vi "CreateClass.vi"(0 "ClassWriterGOOP400.lvclass":refnum<class "ClassWriterGOOP400.lvclass">, 1 "ProjectTreePosition(String or Project Item Ref)":variant, 2 "CreateClassData":T1, 5 "error in (no error)":errorcluster, 6 "KeepLvClassRefOpen(False)":bool, 7 "HeaderToApply (take from VIRef or /use 2D-8bit header, Ignored if not wired)":variant) -> (14 "ClassWriterGOOP400.lvclass":refnum<class "ClassWriterGOOP400.lvclass">, 15 "LVClassLibraryRefnum":refnum<vi>, 16 "TemplateVersionUsed":string, 19 "error out":errorcluster)   [LabVIEW 2020, in "ClassWriterGOOP400.lvclass"]
uses:
  ClassWriterGOOP400.lvclass
  Provider_BaseClassInterface/CreateClassData.ctl
  Common/LvClass_class/GDSLvCLass_ClassSettingsType.ctl
  Common/LvClass_class/GDSLvClass_PlugIn.ctl
  Common/LvClass_class/GDSLvClass_PlugInTypes.ctl
  EndevoG4ProviderName.ctl
  Provider_BaseClassInterface/ClassWriter_class/ClassWriter.lvclass
  Provider_LvNativeClass/ClassWriterNative_class/ClassWriterNative.lvclass
  Common/InterfaceLibrary/InterfaceLibrary.lvlib
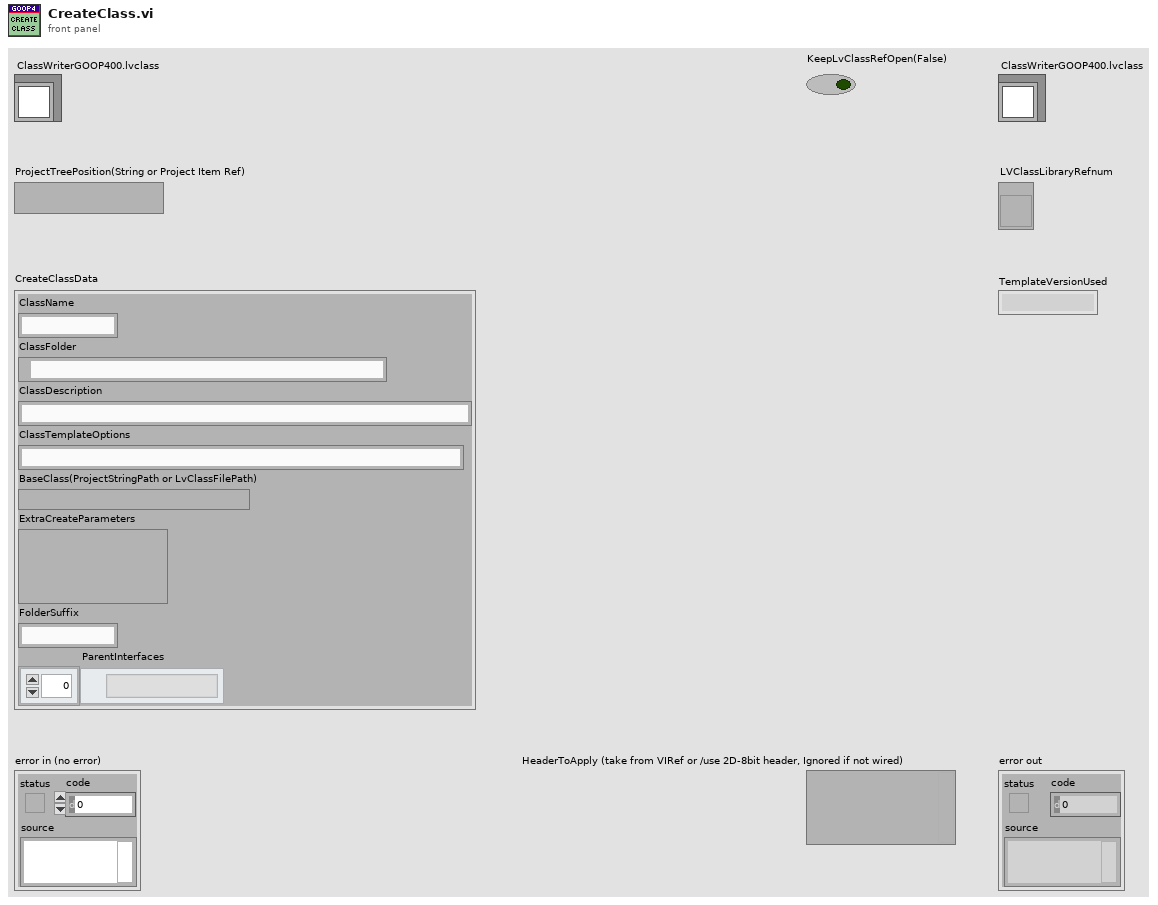
[diagram p1: front panel]
types:
  T1 = typedef "ClassWriter.lvclass/CreateClassData.ctl" = cluster{"ClassName":string, "ClassFolder":path, "ClassDescription":string, "ClassTemplateOptions":string, "BaseClass(ProjectStringPath or LvClassFilePath)":variant, "ExtraCreateParameters":variant, "FolderSuffix":string, "ParentInterfaces":path[]}
  T2 = typedef "GDSLvCLass_ClassSettingsType.ctl" = cluster{"ClassProviderName":string, "ClassTemplateUsed":string, "ClassTemplateVersion":string, "ClassDescription":string, "PlugIns":T3[], "ConnectorPanePattern":string}
  T3 = typedef "GDSLvClass_PlugIn.ctl" = cluster{"Type":T4, "ID":string, "Version":string, "Path":path, "Name":string, "Data":variant}
  T4 = typedef "GDSLvClass_PlugInTypes.ctl" = enum16{"DesignPattern", "MethodTypes"}
  T5 = cluster{"SubClass":bool, "ClassTemplateFiles":path[], "ClassName":string, "ClassFolder":path, "VIs":refnum<vi>[], "TemplateFolder":path, "ViSubDirs":string[], "TemplateName":string, "BaseClassFolder":path, "RootBaseClassFolder":path, "LvClassPath":path, "ClassRefnum":refnum<vi>, "ProjectRefnum":refnum<vi>, "LvClassFolderPath":path, "BaseClassName":string, "ClassItems":refnum<vi>[], "ViLocked":bool[], "ProjectItemOwner":refnum<vi>, "DeleteFiles":path[], "VIsBefore":refnum<vi>[], "BaseClassPath":path, "BaseConstructorBase":path, "TemplBaseConstructorBase":path, "TemplatePath":path, "TemplateVersion":string, "TemplateParentClass":refnum<vi>, "App":refnum<vi>, "Parent Class":refnum<vi>, "ParentVIs":refnum<vi>[], "TempClass":refnum<vi>, "ClassSettings":T2}
  T6 = typedef "EndevoG4ProviderName.ctl" = enum16{"EndevoGOOP400"}
  T7 = enum32{"invalid scope", "public", "private", "protected"}
  T8 = enum32{"invalid lock state", "Not Locked", "Locked (No Password)", "Password-protected"}
  T9 = typedef "ClassWriter.lvclass/TemplateSettings.ctl" = cluster{"CommonClassTemplate":bool, "DynamicDispatch":enum8{"False", "True", "Mixed"}, "MustOverride":enum8{"False", "True", "Mixed"}, "MustCallParent":enum8{"False", "True", "Mixed"}, "OnlyNormalMethod":bool, "OnlyPublic":bool}
  T10 = typedef "Scripting_ConnectorPanePatternType.ctl" = u16
  T11 = typedef "GOOP400_Options.ctl" = cluster{"FlatFolderStructure":bool}
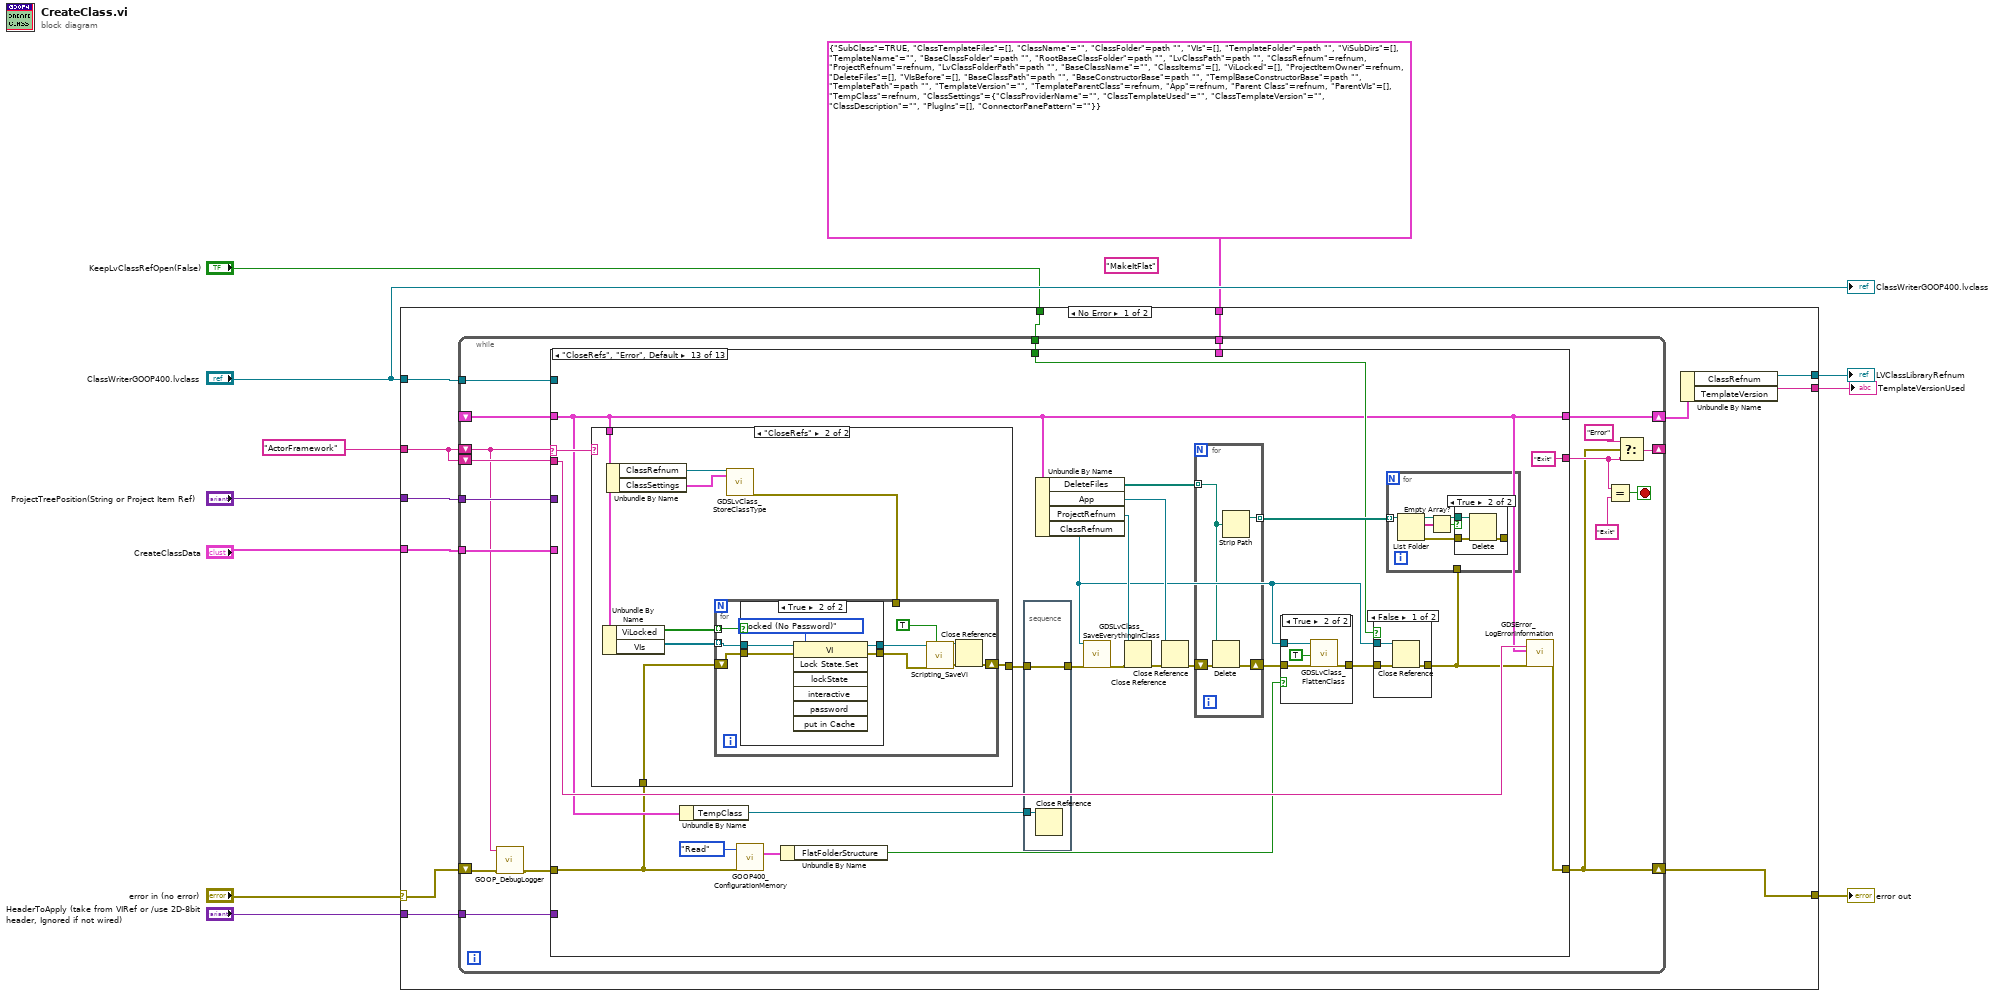
[diagram p0: block diagram]
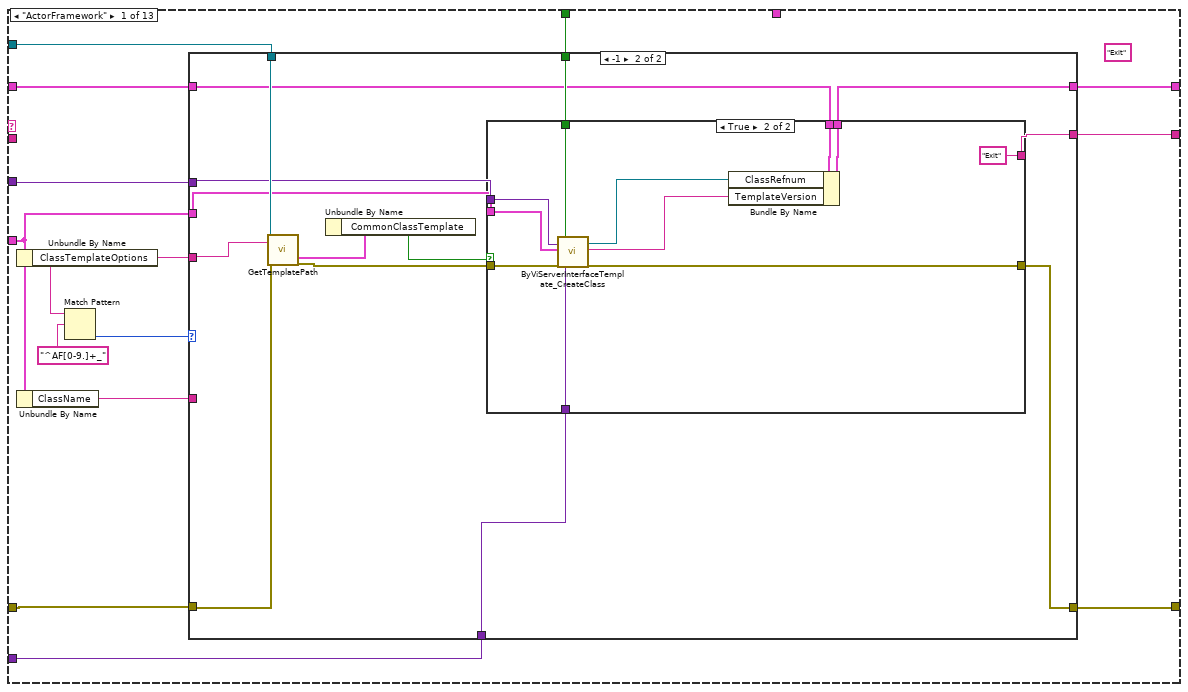
[diagram p2: hidden frame]
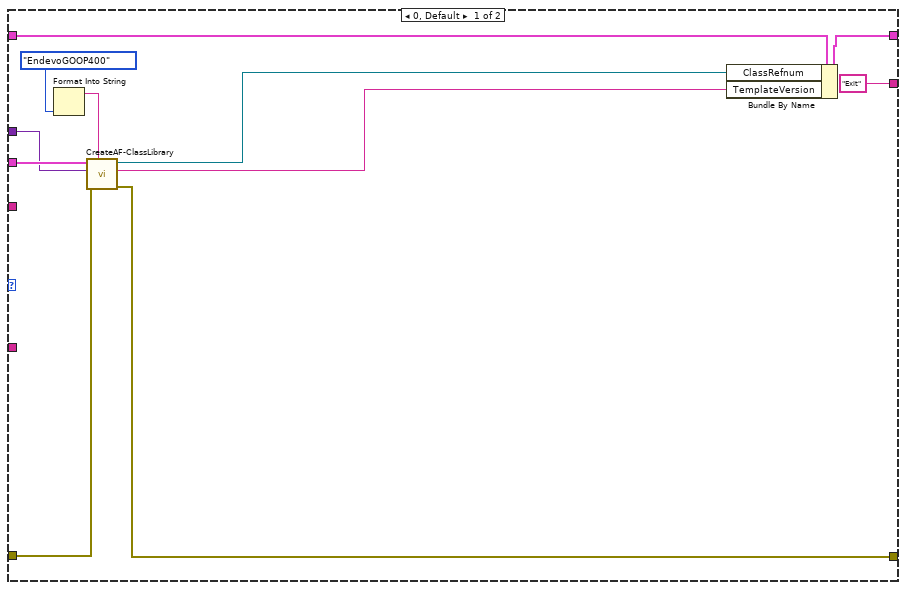
[diagram p3: hidden frame]
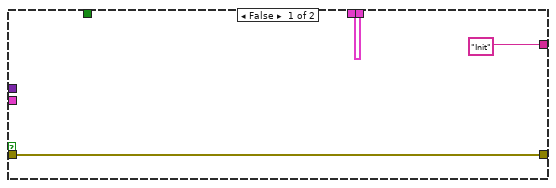
[diagram p4: hidden frame]
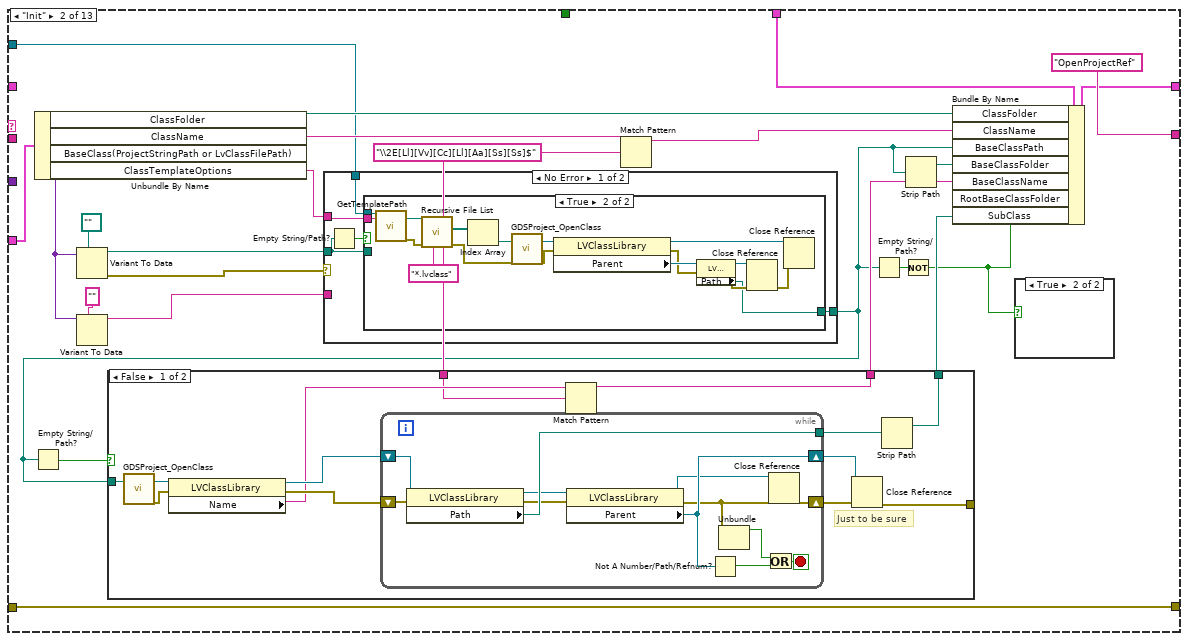
[diagram p5: hidden frame]
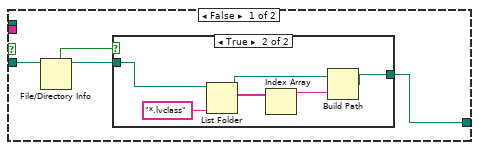
[diagram p6: hidden frame]
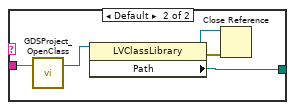
[diagram p9: hidden frame]
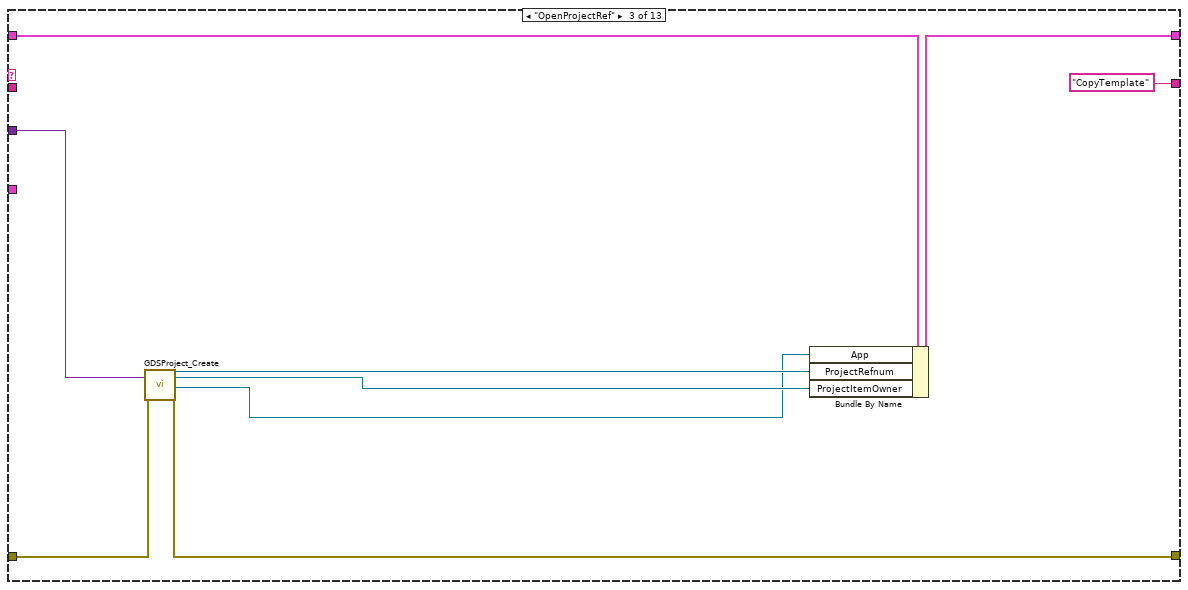
[diagram p12: hidden frame]
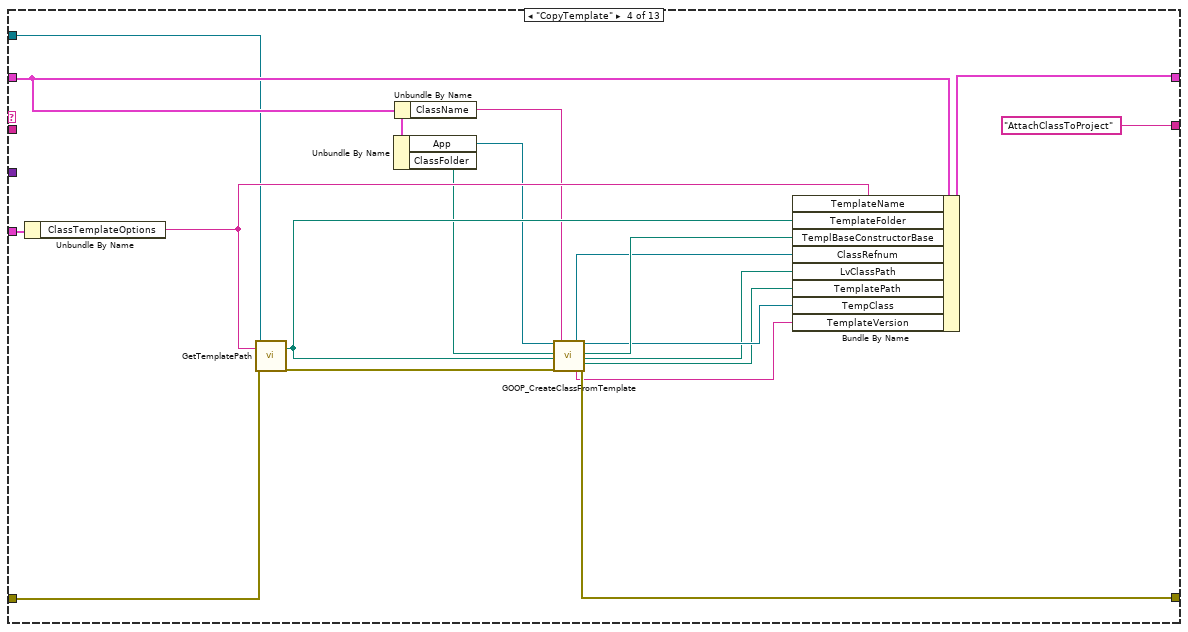
[diagram p13: hidden frame]
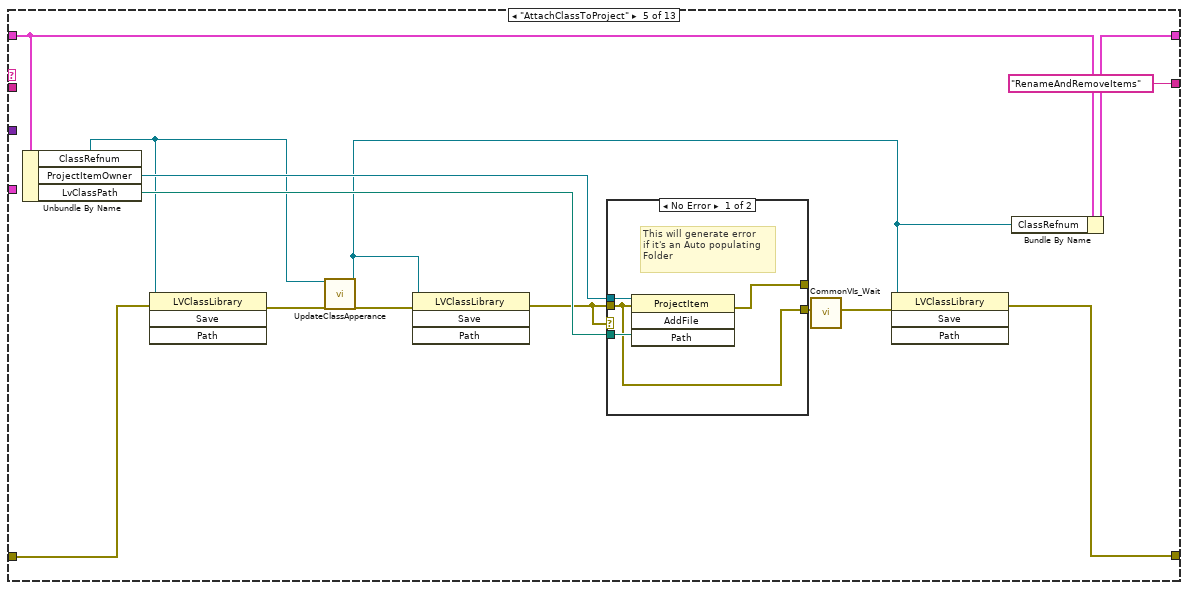
[diagram p14: hidden frame]
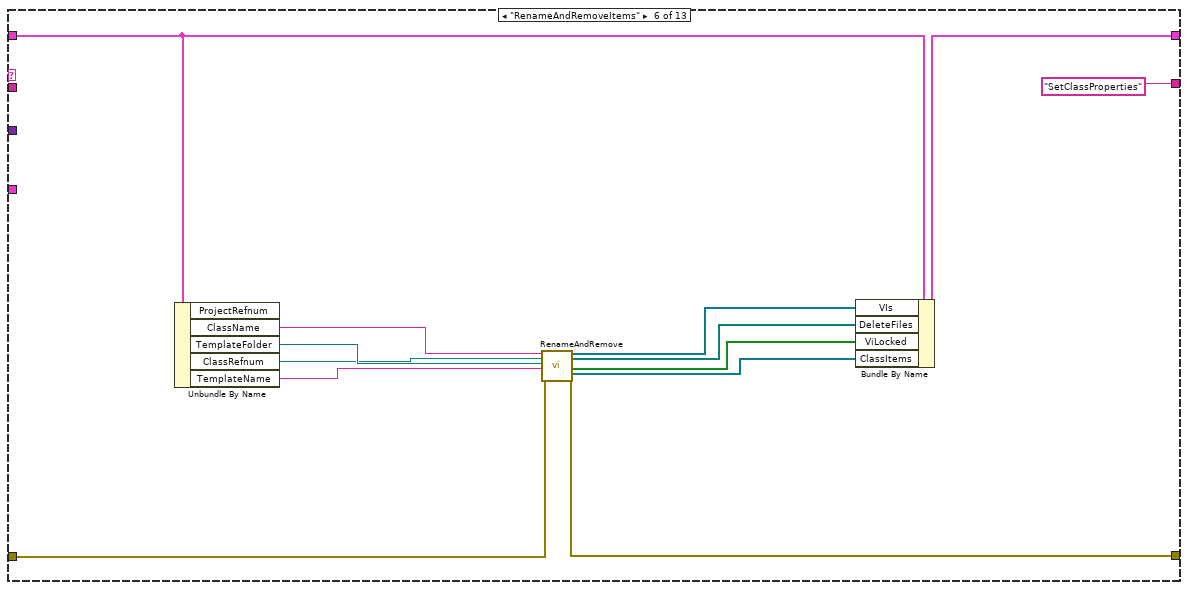
[diagram p16: hidden frame]
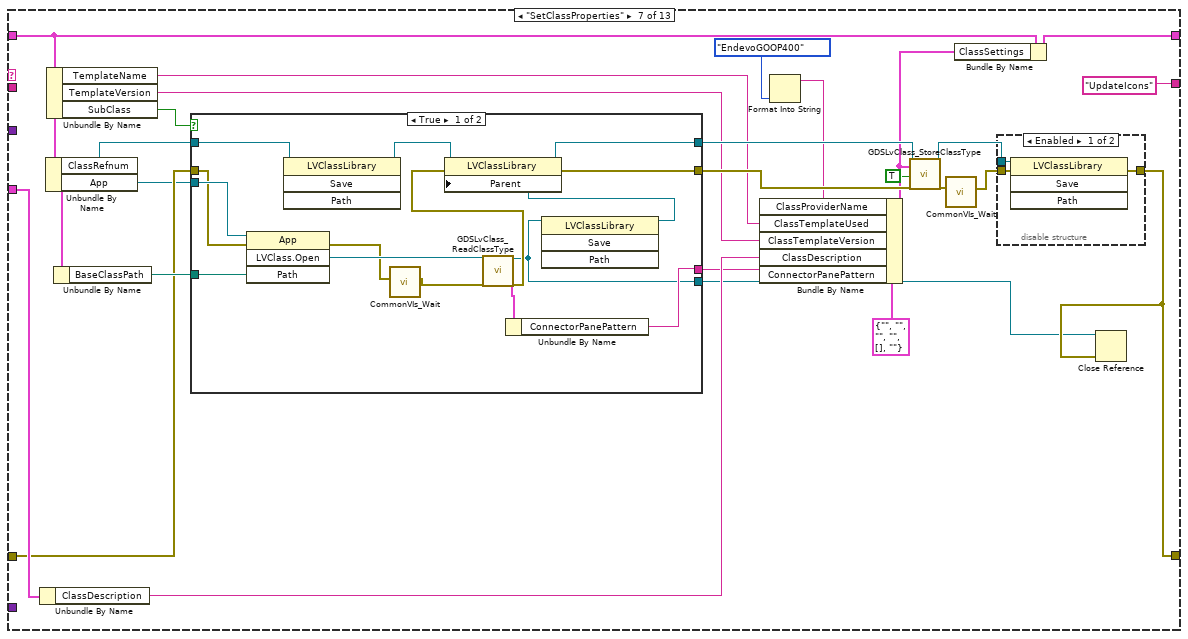
[diagram p17: hidden frame]
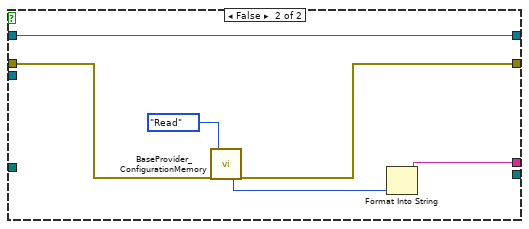
[diagram p19: hidden frame]
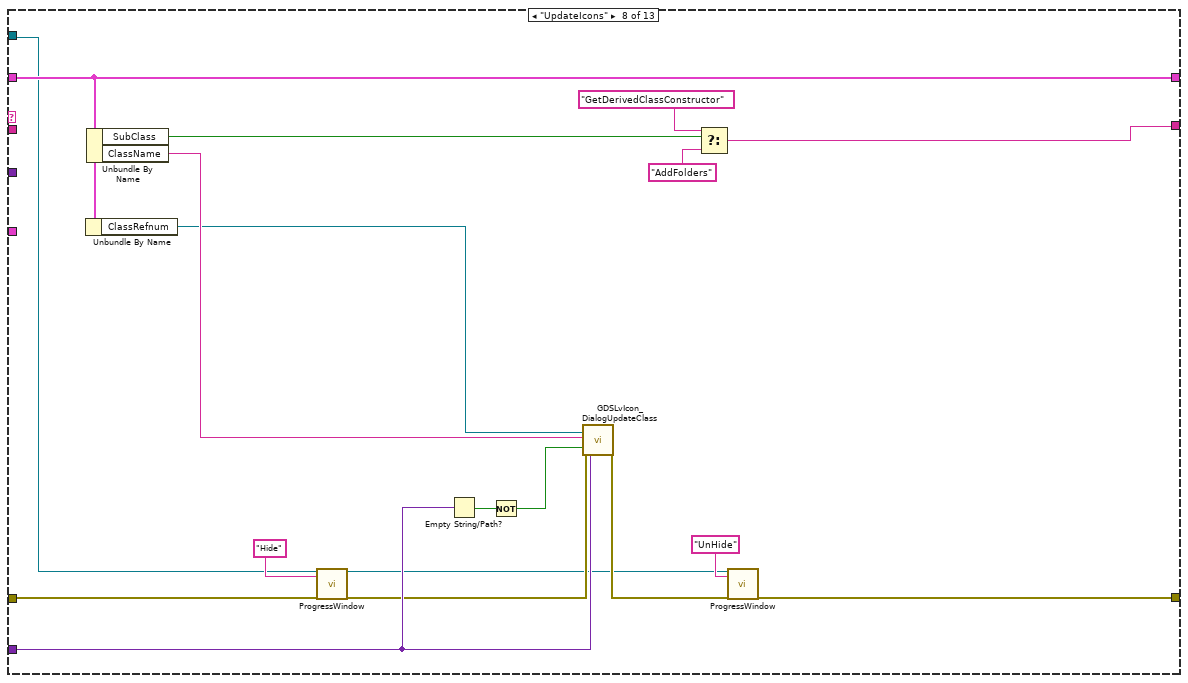
[diagram p20: hidden frame]
diagram:
  (unwired) "MakeItFlat"
  n1 = case shown="No Error" "error in (no error)" {
    selector: "error in (no error)" -> [w13 w610]
    tunnel: [w23 w610] -> w11
    tunnel: "ProjectTreePosition(String or Project Item Ref)" -> [w22 _]
    tunnel: "CreateClassData" -> [w21 _]
    tunnel: "ClassWriterGOOP400.lvclass" -> [w20 _]
    tunnel: "HeaderToApply (take from VIRef or /use 2D-8bit header, Ignored if not wired)" -> [w19 _]
    tunnel: "KeepLvClassRefOpen(False)" -> [w18 _]
    tunnel: [w17 _] -> w4
    tunnel: [w16 _] -> w3
    tunnel: T5 {"SubClass"=TRUE, "ClassTemplateFiles"=[], "ClassName"="", "ClassFolder"=path "", "VIs"=[], "TemplateFolder"=path "", "ViSubDirs"=[], "TemplateName"="", "BaseClassFolder"=path "", "RootBaseClassFolder"=path "", "LvClassPath"=path "", "ClassRefnum"=refnum, "ProjectRefnum"=refnum, "LvClassFolderPath"=path "", "BaseClassName"="", "ClassItems"=[], "ViLocked"=[], "ProjectItemOwner"=refnum, "DeleteFiles"=[], "VIsBefore"=[], "BaseClassPath"=path "", "BaseConstructorBase"=path "", "TemplBaseConstructorBase"=path "", "TemplatePath"=path "", "TemplateVersion"="", "TemplateParentClass"=refnum, "App"=refnum, "Parent Class"=refnum, "ParentVIs"=[], "TempClass"=refnum, "ClassSettings"={"ClassProviderName"="", "ClassTemplateUsed"="", "ClassTemplateVersion"="", "ClassDescription"="", "PlugIns"=[], "ConnectorPanePattern"=""}} ("output cluster") -> [w15 _]
    tunnel: "ActorFramework" -> [w12 _]
    frame No Error {
      n2 = while {
        shift-right: [w33] -> w23
        shift-left: w13 -> [w26]
        shift-right: [w37] -> _
        shift-left: w12 -> [w24]
        shift-right: [w40] -> w14
        shift-left: _ -> [w41]
        tunnel: w15 -> [w35]
        tunnel: w22 -> [w32]
        tunnel: w21 -> [w31]
        tunnel: w20 -> [w30]
        shift-left: w12 -> [w29]
        tunnel: w19 -> [w28]
        tunnel: w18 -> [w27]
        stop <- w38 stop-if-true
        n3 = call "GOOP_DebugLogger.vi"("error in (no error)"=w26, "State"=w24) -> ("error out"=w25:errorcluster)  [unwired: 7 in, 2 out]
        n4 = case shown="\"CloseRefs\", \"Error\", Default" w24 {
          selector: w24 -> [_ _ _ _ _ _ _ _ _ _ _ _ w558]
          tunnel: w41 -> [w55 _ w190 w208 w223 w238 w256 w306 w328 w337 w450 w516 w547]
          tunnel: [w54 w115 w189 w210 w222 w240 w245 w306 w329 w337 w450 w516 w547] -> w40
          tunnel: w25 -> [w50 w118 w188 w204 w217 w235 w257 w299 w325 w351 w471 w518 w542]
          tunnel: [w49 w118 w186 w199 w213 w236 w247 w296 w311 w335 w451 w519 w556] -> w33
          tunnel: [w53 "OpenProjectRef" "CopyTemplate" "AttachClassToProject" "RenameAndRemoveItems" "SetClassProperties" "UpdateIcons" w308 "UpdateVIs" ("t") "AddFolders" "AddFolders" "CloseRefs" "Exit"] -> w34
          tunnel: w35 -> [_ w112 _ _ _ _ _ _ _ _ _ _ _]
          tunnel: w32 -> [w48 _ w187 _ _ _ _ _ _ _ _ _ _]
          tunnel: w31 -> [w46 w111 _ w207 _ _ w263 _ _ _ _ w507 _]
          tunnel: w30 -> [w44 w97 _ w205 _ _ _ w293 _ _ _ _ _]
          tunnel: w29 -> [_ _ _ _ _ _ _ _ _ _ _ _ w555]
          tunnel: w28 -> [w42 _ _ _ _ _ _ w304 _ _ _ _ _]
          tunnel: w27 -> [w43 _ _ _ _ _ _ _ _ _ _ _ w552]
          frame "ActorFramework" {
            (unwired) "Exit"
            n5 = Unbundle By Name(w46) -> ("ClassTemplateOptions"=w47:string)
            n6 = Unbundle By Name(w46) -> ("ClassName"=w45:string)
            n7 = Match Pattern(string=w47, regular expression="^AF[0-9.]+_") -> (offset past match=w51:i32)  [unwired: 1 in, 3 out]
            n8 = case shown="-1" w51 {
              tunnel: w55 -> [w66 w73]
              tunnel: [w65 w72] -> w54
              tunnel: ["Exit" w80] -> w53
              tunnel: w46 -> [w63 w70]
              tunnel: w50 -> [w62 w79]
              tunnel: [w61 w75] -> w49
              tunnel: w48 -> [w58 w71]
              tunnel: w47 -> [_ w77]
              tunnel: w45 -> [_ _]
              tunnel: w44 -> [_ w78]
              tunnel: w43 -> [_ w74]
              tunnel: w42 -> [_ w69]
              frame 0, Default {
                n9 = Format Into String(EndevoG4ProviderName."EndevoGOOP400" ("ProviderName")) -> (resulting string=w60:string)  [unwired: 3 in, 1 out]
                n10 = call "CreateAF-ClassLibrary.vi"("Providername"=w60, "error in (no error)"=w62, "ProjectTreePosition(String or Project Item Ref)"=w58, "CreateClassData"=w63) -> ("error out"=w61:errorcluster, "TemplateVersionUsed"=w59:string, "LVClassLibraryRefnum"=w56:refnum<vi>)  [unwired: 5 in]
                n11 = Bundle By Name(cluster=w66, "ClassRefnum"=w56, "TemplateVersion"=w59) -> (w65:T5)
              }
              frame -1 {
                n12 = call-dynamic "GetTemplatePath.vi"("reference in"=w78, "ClassTemplateSubDirectory"=w77, "error in (no error)"=w79) -> ("TemplateSettings"=w68:T9, "error out"=w76:errorcluster)  [unwired: 12 in, 3 out]
                n13 = Unbundle By Name(w68) -> ("CommonClassTemplate"=w67:bool)
                n14 = case shown="True" w67 {
                  tunnel: ["Init" "Exit"] -> w80
                  tunnel: w76 -> [w82 w91]
                  tunnel: [w82 w90] -> w75
                  tunnel: w74 -> [_ w89]
                  tunnel: w73 -> [w81 w88]
                  tunnel: [w81 w87] -> w72
                  tunnel: w71 -> [_ w86]
                  tunnel: w70 -> [_ w85]
                  tunnel: w69 -> [_ w84]
                  frame False {
                  }
                  frame True {
                    n15 = call "ByViServerInterfaceTemplate_CreateClass.vi"("ProjectTreePosition(String or Project Item Ref)"=w86, "CreateClassData"=w85, "error in (no error)"=w91, "KeepLvClassRefOpen(False)"=w89, "HeaderToApply (take from VIRef or /use 2D-8bit header, Ignored if not wired)"=w84) -> ("LVClassLibraryRefnum"=w93:refnum<vi>, "TemplateVersionUsed"=w92:string, "error out"=w90:errorcluster)  [unwired: 12 in]
                    n16 = Bundle By Name(cluster=w88, "ClassRefnum"=w93, "TemplateVersion"=w92) -> (w87:T5)
                  }
                }
              }
            }
          }
          frame "Init" {
            w108 = "\\2E[Ll][Vv][Cc][Ll][Aa][Ss][Ss]$" ("regular expression")
            n17 = Unbundle By Name(w111) -> ("ClassFolder"=w105:path, "ClassName"=w104:string, "BaseClass(ProjectStringPath or LvClassFilePath)"=w110:variant, "ClassTemplateOptions"=w96:string)
            n18 = Variant To Data(type=path "" ("path"), Variant=w110) -> (data=w100:path, error out=w99:errorcluster)  [unwired: 1 in]
            n19 = Variant To Data(type="" ("regular expression"), Variant=w110) -> (data=w98:string)  [unwired: 1 in, 1 out]
            n20 = case shown="No Error" w99 {
              tunnel: [w123 w152] -> w95
              tunnel: w98 -> [_ w153]
              tunnel: w100 -> [w122 _]
              tunnel: w96 -> [w119 _]
              tunnel: w97 -> [w120 _]
              frame No Error {
                n21 = Empty String/Path?(string/path=w122) -> (empty?=w121:bool)
                n22 = case shown="True" w121 {
                  tunnel: [w127 w135] -> w123
                  tunnel: w122 -> [w124 _]
                  tunnel: w120 -> [_ w137]
                  tunnel: w119 -> [_ w136]
                  frame False {
                    n23 = File/Directory Info(path=w124) -> (path out=w125:path, directory=w126:bool)  [unwired: 1 in, 5 out]
                    n24 = case shown="True" w126 {
                      tunnel: [w128 w130] -> w127
                      tunnel: w125 -> [w128 w129]
                      frame False {
                      }
                      frame True {
                        n25 = List Folder(path=w129, pattern="*.lvclass") -> (path out=w131:path, filenames=w133:string[])  [unwired: 2 in, 2 out]
                        n26 = Index Array(array=w133) -> (element=w132:string)  [unwired: 1 in]
                        n27 = Build Path(base path=w131, name or relative path=w132) -> (appended path=w130:path)
                      }
                    }
                  }
                  frame True {
                    n28 = call-dynamic "GetTemplatePath.vi"("reference in"=w137, "ClassTemplateSubDirectory"=w136) -> ("FolderPathOut"=w149:path, "error out"=w139:errorcluster)  [unwired: 13 in, 3 out]
                    n29 = call <vilib>:"Recursive File List.vi"("pattern"="*.lvclass", "error in (no error)"=w139, "Folder Path"=w149) -> ("error out"=w138:errorcluster, "All Files in Dir"=w150:path[])  [unwired: 4 in, 3 out]
                    n30 = Index Array(array=w150) -> (element=w148:path)  [unwired: 1 in]
                    n31 = call "GDSProject_OpenClass.vi"("ClassPath(FilePath/ProjectTreePath/LvCLassRef)"=w148, "error IO"=w138) -> ("LVClass.Open"=w146:refnum<vi>, "error out"=w147:errorcluster)  [unwired: 15 in, 1 out]
                    n32 = property class="LVClassLibrary"(reference=w146, error in=w147) -> (reference out=w140:refnum<vi>, error out=w144:errorcluster, "Parent"=w145:refnum<vi>)
                    n33 = property class="LVClassLibrary"(reference=w145, error in=w144) -> (reference out=w142:refnum<vi>, error out=w143:errorcluster, "Path"=w135:path)
                    n34 = Close Reference(reference=w142, error in (no error)=w143) -> (error out=w141:errorcluster)
                    n35 = Close Reference(reference=w140, error in (no error)=w141) -> ()  [unwired: 1 out]
                  }
                }
              }
              frame Error {
                n36 = case shown="\"\"" w153 {
                  tunnel: w153 -> [_ w158]
                  tunnel: [_ w154] -> w152
                  frame "" {
                  }
                  frame Default {
                    n37 = call "GDSProject_OpenClass.vi"("ClassPath(FilePath/ProjectTreePath/LvCLassRef)"=w158) -> ("LVClass.Open"=w157:refnum<vi>)  [unwired: 16 in, 2 out]
                    n38 = property class="LVClassLibrary"(reference=w157) -> (reference out=w155:refnum<vi>, error out=w156:errorcluster, "Path"=w154:path)  [unwired: 1 in]
                    n39 = Close Reference(reference=w155, error in (no error)=w156) -> ()  [unwired: 1 out]
                  }
                }
              }
            }
            n40 = Empty String/Path?(string/path=w95) -> (empty?=w106:bool)
            n41 = case shown="False" w106 {
              tunnel: [w168 _] -> w109
              tunnel: w108 -> [w162 _]
              tunnel: [w161 _] -> w107
              tunnel: w95 -> [w160 _]
              tunnel: [w159 _] -> _
              frame False {
                # "Just to be sure"
                n42 = call "GDSProject_OpenClass.vi"("ClassPath(FilePath/ProjectTreePath/LvCLassRef)"=w160) -> ("LVClass.Open"=w165:refnum<vi>, "error out"=w167:errorcluster)  [unwired: 16 in, 1 out]
                n43 = property class="LVClassLibrary"(reference=w165, error in=w167) -> (reference out=w164:refnum<vi>, error out=w166:errorcluster, "Name"=w163:string)
                n44 = while {
                  shift-right: [w179] -> w171
                  shift-left: w166 -> [w174]
                  shift-right: [w180] -> w170
                  shift-left: w164 -> [w182]
                  tunnel: [w181] -> w169
                  stop <- w176 stop-if-true
                  n45 = property class="LVClassLibrary"(reference=w182, error in=w174) -> (reference out=w172:refnum<vi>, error out=w173:errorcluster, "Path"=w181:path)
                  n46 = property class="LVClassLibrary"(reference=w172, error in=w173) -> (reference out=w175:refnum<vi>, error out=w179:errorcluster, "Parent"=w180:refnum<vi>)
                  n47 = Not A Number/Path/Refnum?(number/path/refnum=w180) -> (NaN/Path/Refnum?=w177:bool)
                  n48 = Unbundle(w179) -> ("status"=w178:bool)  [unwired: 2 out]
                  n49 = Or(x=w178, y=w177) -> (x .or. y?=w176:bool)
                  n50 = Close Reference(reference=w175) -> ()  [unwired: 1 in, 1 out]
                }
                n51 = Match Pattern(string=w163, regular expression=w162) -> (before substring=w161:string)  [unwired: 1 in, 3 out]
                n52 = Close Reference(reference=w170, error in (no error)=w171) -> (error out=w159:errorcluster)
                n53 = Strip Path(path=w169) -> (stripped path=w168:path)  [unwired: 1 out]
              }
              frame True {
              }
            }
            n54 = Match Pattern(string=w104, regular expression=w108) -> (before substring=w116:string)  [unwired: 1 in, 3 out]
            n55 = Empty String/Path?(string/path=w95) -> (empty?=w102:bool)
            n56 = Not(x=w102) -> (.not. x?=w101:bool)
            n57 = Strip Path(path=w95) -> (stripped path=w103:path)  [unwired: 1 out]
            n58 = Bundle By Name(cluster=w112, "ClassFolder"=w105, "ClassName"=w116, "BaseClassPath"=w95, "BaseClassFolder"=w103, "BaseClassName"=w107, "RootBaseClassFolder"=w109, "SubClass"=w101) -> (w115:T5)
            n59 = case shown="True" w101 {
              frame False {
              }
              frame True {
              }
            }
          }
          frame "OpenProjectRef" {
            n60 = call "GDSProject_Create.vi"("ProjectTreePosition(String or Project Item Ref)"=w187, "error in (no error)"=w188) -> ("Project Refnum"=w184:refnum<vi>, "Project Item"=w185:refnum<vi>, "App"=w183:refnum<vi>, "error out"=w186:errorcluster)  [unwired: 13 in, 1 out]
            n61 = Bundle By Name(cluster=w190, "App"=w183, "ProjectRefnum"=w184, "ProjectItemOwner"=w185) -> (w189:T5)
          }
          frame "CopyTemplate" {
            n62 = Unbundle By Name(w207) -> ("ClassTemplateOptions"=w206:string)
            n63 = call-dynamic "GetTemplatePath.vi"("reference in"=w205, "ClassTemplateSubDirectory"=w206, "error in (no error)"=w204) -> ("FolderPathOut"=w202:path, "error out"=w203:errorcluster)  [unwired: 12 in, 3 out]
            n64 = Unbundle By Name(w208) -> ("App"=w200:refnum<vi>, "ClassFolder"=w196:path)
            n65 = Unbundle By Name(w208) -> ("ClassName"=w192:string)
            n66 = call "GOOP_CreateClassFromTemplate.vi"("Application in"=w200, "ClassFolder"=w196, "TeplateClassFolder"=w202, "error in (no error)"=w203, "ClassName"=w192) -> ("NewClassRef"=w193:refnum<vi>, "TemplateClassVersionString"=w194:string, "TemplateClassRef"=w198:refnum<vi>, "TemplateClassConstructorPath(*Create, *Init)"=w201:path, "NewClassPath"=w197:path, "TemplateClassPath"=w195:path, "error out"=w199:errorcluster)  [unwired: 7 in, 1 out]
            n67 = Bundle By Name(cluster=w208, "TemplateName"=w206, "TemplateFolder"=w202, "TemplBaseConstructorBase"=w201, "ClassRefnum"=w193, "LvClassPath"=w197, "TemplatePath"=w195, "TempClass"=w198, "TemplateVersion"=w194) -> (w210:T5)
          }
          frame "AttachClassToProject" {
            n68 = Unbundle By Name(w223) -> ("ClassRefnum"=w216:refnum<vi>, "ProjectItemOwner"=w224:refnum<vi>, "LvClassPath"=w220:path)
            n69 = invoke class="LVClassLibrary" method="Save"(reference=w216, error in=w217) -> (error out=w218:errorcluster)  [unwired: 2 in, 3 out]
            n70 = call "UpdateClassApperance.vi"("ClassRefIn"=w216, "error in (no error)"=w218) -> ("ClassRefOut"=w211:refnum<vi>, "error out"=w215:errorcluster)  [unwired: 16 in]
            n71 = invoke class="LVClassLibrary" method="Save"(reference=w211, error in=w215) -> (error out=w212:errorcluster)  [unwired: 2 in, 3 out]
            n72 = case shown="No Error" w212 {
              tunnel: w224 -> [w228 _]
              tunnel: w220 -> [w227 _]
              tunnel: [w226 w229] -> w219
              tunnel: w212 -> [w226 w229]
              tunnel: [w225 _] -> _
              frame No Error {
                # "This will generate error\nif it's an Auto populating\nFolder"
                n73 = invoke class="ProjectItem" method="AddFile"(reference=w228, error in=w226, "Path"=w227) -> (error out=w225:errorcluster)  [unwired: 1 in, 3 out]
              }
              frame Error {
              }
            }
            n74 = call "CommonVIs_Wait.vi"("error in"=w219) -> ("error out"=w214:errorcluster)  [unwired: 9 in]
            n75 = invoke class="LVClassLibrary" method="Save"(reference=w211, error in=w214) -> (error out=w213:errorcluster)  [unwired: 2 in, 3 out]
            n76 = Bundle By Name(cluster=w223, "ClassRefnum"=w211) -> (w222:T5)
          }
          frame "RenameAndRemoveItems" {
            n77 = Unbundle By Name(w238) -> ("ClassName"=w242:string, "TemplateFolder"=w239:path, "ClassRefnum"=w237:refnum<vi>, "TemplateName"=w230:string)  [unwired: 1 out]
            n78 = call "RenameAndRemove.vi"("ClassName"=w242, "ClassRefnum"=w237, "TemplateFolder"=w239, "TemplateName"=w230, "error in"=w235) -> ("ViRefsOut"=w241:refnum<vi>[], "DeleteFiles"=w234:path[], "ItemLocked"=w233:bool[], "Items"=w232:refnum<vi>[], "error out"=w236:errorcluster)  [unwired: 10 in]
            n79 = Bundle By Name(cluster=w238, "VIs"=w241, "DeleteFiles"=w234, "ViLocked"=w233, "ClassItems"=w232) -> (w240:T5)
          }
          frame "SetClassProperties" {
            n80 = Unbundle By Name(w263) -> ("ClassDescription"=w260:string)
            n81 = Unbundle By Name(w256) -> ("ClassRefnum"=w258:refnum<vi>, "App"=w252:refnum<vi>)
            n82 = Unbundle By Name(w256) -> ("TemplateName"=w259:string, "TemplateVersion"=w253:string, "SubClass"=w267:bool)
            n83 = Unbundle By Name(w256) -> ("BaseClassPath"=w266:path)
            n84 = case shown="True" w267 {
              tunnel: w258 -> [w275 w292]
              tunnel: [w286 w292] -> w265
              tunnel: w257 -> [w279 w289]
              tunnel: [w285 w288] -> w264
              tunnel: w266 -> [w284 _]
              tunnel: w252 -> [w280 _]
              tunnel: [w281 w290] -> w251
              tunnel: [w273 _] -> w246
              frame True {
                n85 = invoke class="App" method="LVClass.Open"(reference=w280, error in=w279, "Path"=w284) -> (error out=w278:errorcluster, "LVClass.Open"=w283:refnum<vi>)  [unwired: 1 in, 2 out]
                n86 = invoke class="LVClassLibrary" method="Save"(reference=w275) -> (reference out=w274:refnum<vi>)  [unwired: 3 in, 3 out]
                n87 = call "CommonVIs_Wait.vi"("error in"=w278) -> ("error out"=w277:errorcluster)  [unwired: 9 in]
                n88 = call "GDSLvClass_ReadClassType.vi"("Class Refnum In"=w283, "error in (no error)"=w277) -> ("Class Refnum Out"=w273:refnum<vi>, "ClassSettings"=w282:T2, "error out"=w276:errorcluster)  [unwired: 15 in]
                n89 = Unbundle By Name(w282) -> ("ConnectorPanePattern"=w281:string)
                n90 = invoke class="LVClassLibrary" method="Save"(reference=w273) -> (reference out=w272:refnum<vi>)  [unwired: 3 in, 3 out]
                n91 = property class="LVClassLibrary"(reference=w274, error in=w276, "Parent"=w272) -> (reference out=w286:refnum<vi>, error out=w285:errorcluster)
              }
              frame False {
                n92 = call "BaseProvider_ConfigurationMemory.vi"("error in (no error)"=w289, "Action"=enum16{"Read", "Load", "Save", "Set"}."Read") -> ("PatternOut"=w291:T10, "error out"=w288:errorcluster)  [unwired: 11 in, 5 out]
                n93 = Format Into String(w291) -> (resulting string=w290:string)  [unwired: 3 in, 1 out]
              }
            }
            n94 = Format Into String(EndevoG4ProviderName."EndevoGOOP400" ("ProviderName")) -> (resulting string=w261:string)  [unwired: 3 in, 1 out]
            n95 = Bundle By Name(cluster=T2 {"ClassProviderName"="", "ClassTemplateUsed"="", "ClassTemplateVersion"="", "ClassDescription"="", "PlugIns"=[], "ConnectorPanePattern"=""} ("ClassSettings"), "ClassProviderName"=w261, "ClassTemplateUsed"=w259, "ClassTemplateVersion"=w253, "ClassDescription"=w260, "ConnectorPanePattern"=w251) -> (w244:T2)
            n96 = call "GDSLvClass_StoreClassType.vi"("Class Refnum In"=w265, "ClassSettings"=w244, "CheckAndFixConnectorPaneType(False)"=TRUE, "error in (no error)"=w264) -> ("Class Refnum Out"=w250:refnum<vi>, "error out"=w249:errorcluster)  [unwired: 14 in]
            n97 = call "CommonVIs_Wait.vi"("error in"=w249) -> ("error out"=w248:errorcluster)  [unwired: 9 in]
            n98 = Bundle By Name(cluster=w256, "ClassSettings"=w244) -> (w245:T5)
            n99 = disable-structure shown="Enabled" {
              disable-tunnel: [w270 w271] -> w247
              disable-tunnel: w250 -> [w269 _]
              disable-tunnel: w248 -> [w268 w271]
              frame Enabled {
                n100 = invoke class="LVClassLibrary" method="Save"(reference=w269, error in=w268) -> (error out=w270:errorcluster)  [unwired: 2 in, 3 out]
              }
              frame Disabled {
              }
            }
            n101 = Close Reference(reference=w246, error in (no error)=w247) -> ()  [unwired: 1 out]
          }
          frame "UpdateIcons" {
            n102 = Unbundle By Name(w306) -> ("ClassRefnum"=w305:refnum<vi>)
            n103 = Unbundle By Name(w306) -> ("SubClass"=w310:bool, "ClassName"=w307:string)
            n104 = call-dynamic "ProgressWindow.vi"("ClassWriter in"=w293, "Message(Exit)"="Hide", "error in (no error)"=w299) -> ("ClassWriter out"=w294:refnum<class "ClassWriterGOOP400.lvclass">, "error out"=w298:errorcluster)  [unwired: 15 in]
            n105 = Empty String/Path?(string/path=w304) -> (empty?=w303:bool)
            n106 = Not(x=w303) -> (.not. x?=w302:bool)
            n107 = call "GDSLvIcon_DialogUpdateClass.vi"("ClassPath(FilePath/ProjectTreePath/LvCLassRef)"=w305, "ClassName"=w307, "AutoUpdate"=w302, "error in (no error)"=w298, "HeaderToApply (take from VIRef or /use 2D-8bit header, Ignored if not wired)"=w304) -> ("error out"=w297:errorcluster)  [unwired: 11 in, 3 out]
            n108 = Select(t="GetDerivedClassConstructor", s=w310, f="AddFolders") -> (s? t:f=w308:string)
            n109 = call-dynamic "ProgressWindow.vi"("ClassWriter in"=w294, "Message(Exit)"="UnHide", "error in (no error)"=w297) -> ("error out"=w296:errorcluster)  [unwired: 15 in, 1 out]
          }
          frame "GetDerivedClassConstructor" {
            # "USE BASE CLASS PATH"
            n110 = Unbundle By Name(w328) -> ("ClassRefnum"=w326:refnum<vi>)
            n111 = property class="LVClassLibrary"(reference=w326, error in=w325) -> (error out=w322:errorcluster, "Parent"=w314:refnum<vi>)  [unwired: 1 out]
            n112 = property class="LVClassLibrary"(reference=w314, error in=w322) -> (reference out=w313:refnum<vi>, error out=w312:errorcluster, "Path"=w320:path)
            n113 = Strip Path(path=w320) -> (stripped path=w319:path)  [unwired: 1 out]
            n114 = call <vilib>:"Recursive File List.vi"("pattern"="*_Create.vi", "Treat LLBs as Folders?"=TRUE, "Folder Path"=w319) -> ("All Files in Dir"=w317:path[], "dup Folder Path"=w315:path)  [unwired: 4 in, 3 out]
            n115 = Close Reference(reference=w313, error in (no error)=w312) -> (error out=w311:errorcluster)
            n116 = Array Size(array=w317) -> (size(s)=w318:i32)
            n117 = case shown="Default" w318 {
              tunnel: w317 -> [w330 _]
              tunnel: [w330 w331] -> w316
              tunnel: w315 -> [_ w332]
              frame Default {
              }
              frame 0 {
                n118 = call <vilib>:"Recursive File List.vi"("pattern"="*_Init.vi", "Treat LLBs as Folders?"=TRUE, "Folder Path"=w332) -> ("All Files in Dir"=w331:path[])  [unwired: 4 in, 4 out]
              }
            }
            n119 = Index Array(array=w316) -> (element=w321:path)  [unwired: 1 in]
            n120 = Bundle By Name(cluster=w328, "BaseConstructorBase"=w321) -> (w329:T5)
          }
          frame "UpdateVIs" {
            (unwired) "AnyProtectedAttributesToUpdate?"
            # "This is a sub class, replace all BaseClass References with Select base class.\nIf base not equal to root, also replace BaseClass ObjectRef with Root-Base ObjectRef"
            n121 = Unbundle By Name(w337) -> ("TemplBaseConstructorBase"=w349:path, "BaseConstructorBase"=w348:path)
            n122 = Unbundle By Name(w337) -> ("VIs"=w352:refnum<vi>[])
            n123 = call "CreateVINamesToReplace.vi"("Foldername"="utils" ("name or relative path"), "NewVIName"="_New.vi" ("string"), "BaseConstructorBase"=w348, "TemplBaseConstructorBase"=w349) -> ("NewVIName"=w345:path, "OldVIName"=w346:path)  [unwired: 5 in]
            n124 = call "CreateVINamesToReplace.vi"("NewVIName"="_Init.vi" ("string"), "BaseConstructorBase"=w348, "TemplBaseConstructorBase"=w349) -> ("NewVIName"=w341:path, "OldVIName"=w342:path)  [unwired: 6 in]
            n125 = call "CreateVINamesToReplace.vi"("NewVIName"="_CleanUp.vi" ("string"), "BaseConstructorBase"=w348, "TemplBaseConstructorBase"=w349) -> ("NewVIName"=w338:path, "OldVIName"=w339:path)  [unwired: 6 in]
            n126 = for {
              shift-right: [w378] -> w335
              shift-left: w351 -> [w375]
              tunnel: w352 -> [w369] mode=indexing
              tunnel: w349 -> [w377]
              tunnel: w348 -> [w376]
              tunnel: w346 -> [w368]
              tunnel: w345 -> [w367]
              tunnel: w342 -> [w361]
              tunnel: w341 -> [w360]
              tunnel: w339 -> [w356]
              tunnel: w338 -> [w355]
              n127 = property class="VI"(reference=w369) -> ("Name"=w354:string)  [unwired: 1 in, 2 out]
              n128 = Match Pattern(string=w354, regular expression="_Create.vi") -> (offset past match=w374:i32)  [unwired: 1 in, 3 out]
              n129 = Match Pattern(string=w354, regular expression="_New.vi") -> (offset past match=w372:i32)  [unwired: 1 in, 3 out]
              n130 = Match Pattern(string=w354, regular expression="_Init.vi") -> (offset past match=w365:i32)  [unwired: 1 in, 3 out]
              n131 = Match Pattern(string=w354, regular expression="_CleanUp.vi") -> (offset past match=w358:i32)  [unwired: 1 in, 3 out]
              n132 = Greater Or Equal To 0?(x=w374) -> (x >= 0?=w363:bool)
              n133 = Greater Or Equal To 0?(x=w372) -> (x >= 0?=w371:bool)
              n134 = Greater Or Equal To 0?(x=w365) -> (x >= 0?=w362:bool)
              n135 = Greater Or Equal To 0?(x=w358) -> (x >= 0?=w357:bool)
              n136 = Compound Arithmetic op=OR(w363, w371, w362, w357) -> (w370:bool)
              n137 = case shown="True" w370 {
                tunnel: w375 -> [w379 w395]
                tunnel: [w379 w394] -> w378
                tunnel: w369 -> [_ w393]
                tunnel: w377 -> [_ w391]
                tunnel: w376 -> [_ w390]
                tunnel: w371 -> [_ w392]
                tunnel: w368 -> [_ w387]
                tunnel: w367 -> [_ w386]
                tunnel: w362 -> [_ w385]
                tunnel: w361 -> [_ w384]
                tunnel: w360 -> [_ w383]
                tunnel: w357 -> [_ w382]
                tunnel: w356 -> [_ w381]
                tunnel: w355 -> [_ w380]
                frame False {
                }
                frame True {
                  n138 = case shown="True" w392 {
                    tunnel: w391 -> [w404 _]
                    tunnel: w390 -> [w402 _]
                    tunnel: [w403 w420] -> w389
                    tunnel: [w401 w419] -> w388
                    tunnel: w387 -> [_ w420]
                    tunnel: w386 -> [_ w419]
                    tunnel: w385 -> [w405 _]
                    tunnel: w384 -> [w400 _]
                    tunnel: w383 -> [w399 _]
                    tunnel: w382 -> [w398 _]
                    tunnel: w381 -> [w397 _]
                    tunnel: w380 -> [w396 _]
                    frame False {
                      n139 = case shown="False" w405 {
                        tunnel: w404 -> [w411 _]
                        tunnel: [w408 w418] -> w403
                        tunnel: w402 -> [w409 _]
                        tunnel: [w410 w417] -> w401
                        tunnel: w400 -> [_ w418]
                        tunnel: w399 -> [_ w417]
                        tunnel: w398 -> [w412 _]
                        tunnel: w397 -> [w407 _]
                        tunnel: w396 -> [w406 _]
                        frame False {
                          n140 = case shown="True" w412 {
                            tunnel: [w414 w416] -> w408
                            tunnel: w411 -> [w414 _]
                            tunnel: [w413 w415] -> w410
                            tunnel: w409 -> [w413 _]
                            tunnel: w407 -> [_ w416]
                            tunnel: w406 -> [_ w415]
                            frame False {
                            }
                            frame True {
                            }
                          }
                        }
                        frame True {
                        }
                      }
                    }
                    frame True {
                    }
                  }
                  n141 = while {
                    tunnel: w395 -> [w435]
                    tunnel: [w432] -> w394
                    tunnel: w393 -> [w424]
                    tunnel: w388 -> [w422]
                    tunnel: w389 -> [w423]
                    i -> [w434]
                    stop <- w433 continue-if-true
                    n142 = File/Directory Info(path=w423) -> (error out=w426:errorcluster)  [unwired: 1 in, 6 out]
                    n143 = File/Directory Info(path=w422) -> (error out=w427:errorcluster)  [unwired: 1 in, 6 out]
                    n144 = Unbundle By Name(w426) -> ("status"=w430:bool)
                    n145 = Unbundle By Name(w427) -> ("status"=w431:bool)
                    n146 = Empty String/Path?(string/path=w422) -> (empty?=w429:bool)
                    n147 = Not Equal?(x=w423, y=w422) -> (x != y?=w421:bool)
                    n148 = Empty String/Path?(string/path=w423) -> (empty?=w428:bool)
                    n149 = Compound Arithmetic op=AND(invert w430, invert w428, invert w431, invert w429, w421) -> (w425:bool)
                    n150 = case shown="True" w425 {
                      tunnel: w435 -> [w436 w448]
                      tunnel: w422 -> [_ w447]
                      tunnel: w423 -> [_ w446]
                      tunnel: w434 -> [_ w444]
                      tunnel: [_ w441] -> w433
                      tunnel: w424 -> [_ w440]
                      tunnel: [w436 w437] -> w432
                      frame False {
                      }
                      frame True {
                        n151 = Build Array(w446) -> (w439:path[])
                        n152 = Build Array(w447) -> (w438:path[])
                        n153 = call "Scripting_ReplaceVisAndControls.vi"("ViRef"=w440, "OldVIsAndControls"=w439, "NewVIsAndControls"=w438, "error in (no error)"=w448) -> ("error out"=w437:errorcluster)  [unwired: 14 in, 1 out]
                        n154 = Unbundle By Name(w437) -> ("status"=w445:bool)  [unwired: 1 out]
                        n155 = Less Or Equal?(x=w444, y=3) -> (x <= y?=w442:bool)
                        n156 = And(x=w442, y=w445) -> (x .and. y?=w441:bool)
                      }
                    }
                  }
                }
              }
            }
            n157 = Unbundle By Name(w337) -> ("TempClass"=w336:refnum<vi>)
            n158 = stacked-sequence {
              tunnel: w336 -> [w353]
              tunnel: w335 -> [_]
              frame #0 {
                n159 = Close Reference(reference=w353) -> ()  [unwired: 1 in, 1 out]
              }
            }
          }
          frame "AnyProtectedAttributesToUpdate?" {
            n160 = Unbundle By Name(w450) -> ("BaseClassFolder"=w468:path)
            n161 = Unbundle By Name(w450) -> ("VIs"=w473:refnum<vi>[])
            n162 = call <vilib>:"Recursive File List.vi"("Folder Path"=w468) -> ("All Files in Dir"=w457:path[])  [unwired: 6 in, 4 out]
            n163 = for {
              tunnel: w473 -> [w501] mode=indexing
              tunnel: [w500] -> w454 mode=indexing
              tunnel: [w498] -> w470 mode=indexing
              n164 = property class="VI"(reference=w501) -> ("Path"=w500:path)  [unwired: 1 in, 2 out]
              n165 = Strip Path(path=w500) -> (name=w499:string)  [unwired: 1 out]
              n166 = To Lower Case(string=w499) -> (all lower case string=w498:string)
            }
            n167 = for {
              tunnel: w457 -> [w486] mode=indexing
              tunnel: [w485] -> w463 mode=indexing
              n168 = Strip Path(path=w486) -> (name=w487:string)  [unwired: 1 out]
              n169 = To Lower Case(string=w487) -> (all lower case string=w485:string)
            }
            n170 = To Lower Case(string="ObjectAttributes.ctl") -> (all lower case string=w467:string)
            n171 = Unbundle By Name(w450) -> ("App"=w449:refnum<vi>)
            n172 = To Lower Case(string="ClassAttributes.ctl") -> (all lower case string=w462:string)
            n173 = Search 1D Array(1D array=w463, element=w467) -> (index of element=w458:i32)  [unwired: 1 in]
            n174 = Search 1D Array(1D array=w463, element=w462) -> (index of element=w456:i32)  [unwired: 1 in]
            n175 = Search 1D Array(1D array=w470, element=w467) -> (index of element=w459:i32)  [unwired: 1 in]
            n176 = Search 1D Array(1D array=w470, element=w462) -> (index of element=w453:i32)  [unwired: 1 in]
            n177 = Greater Or Equal To 0?(x=w456) -> (x >= 0?=w461:bool)
            n178 = Greater Or Equal To 0?(x=w458) -> (x >= 0?=w465:bool)
            n179 = Greater Or Equal To 0?(x=w459) -> (x >= 0?=w466:bool)
            n180 = Greater Or Equal To 0?(x=w453) -> (x >= 0?=w460:bool)
            n181 = And(x=w465, y=w466) -> (x .and. y?=w464:bool)
            n182 = And(x=w461, y=w460) -> (x .and. y?=w455:bool)
            n183 = case shown="True" w464 {
              tunnel: w471 -> [w496 w497]
              tunnel: w454 -> [w495 _]
              tunnel: w457 -> [w493 _]
              tunnel: w459 -> [w491 _]
              tunnel: w458 -> [w490 _]
              tunnel: [w489 w497] -> w452
              tunnel: w449 -> [w488 _]
              frame True {
                n184 = Index Array(array=w495, index=w491) -> (element=w494:path)
                n185 = Index Array(array=w493, index=w490) -> (element=w492:path)
                n186 = call "Scripting_UpdateProtectedClassData.vi"("AppRef"=w488, "error in (no error)"=w496, "NewBaseAttribute"=w492, "BaseAttribute"=w494) -> ("error out"=w489:errorcluster)  [unwired: 6 in, 1 out]
              }
              frame False {
              }
            }
            n187 = case shown="True" w455 {
              tunnel: w454 -> [w483 _]
              tunnel: w457 -> [w481 _]
              tunnel: w453 -> [w479 _]
              tunnel: w456 -> [w478 _]
              tunnel: w452 -> [w477 w484]
              tunnel: [w476 w484] -> w451
              tunnel: w449 -> [w475 _]
              frame True {
                n188 = Index Array(array=w483, index=w479) -> (element=w482:path)
                n189 = Index Array(array=w481, index=w478) -> (element=w480:path)
                n190 = call "Scripting_UpdateProtectedClassData.vi"("AppRef"=w475, "error in (no error)"=w477, "NewBaseAttribute"=w480, "BaseAttribute"=w482) -> ("error out"=w476:errorcluster)  [unwired: 6 in, 1 out]
              }
              frame False {
              }
            }
          }
          frame "AddFolders" {
            n191 = Unbundle By Name(w516) -> ("ClassRefnum"=w517:refnum<vi>)
            n192 = Unbundle By Name(w516) -> ("TemplateName"=w515:string)
            n193 = call "UpdateClassApperance.vi"("ClassRefIn"=w517, "error in (no error)"=w518) -> ("ClassRefOut"=w505:refnum<vi>, "error out"=w510:errorcluster)  [unwired: 16 in]
            n194 = Unbundle By Name(w507) -> ("ParentInterfaces"=w504:path[])
            n195 = call "SetParentInterfaces.vi"("error in"=w510, "Parent Interfaces(ClassRef/Path)"=w504, "Class/InterfaceRefIn"=w505) -> ("error out"=w506:errorcluster)  [unwired: 7 in, 1 out]
            n196 = call "GOOP400_ConfigurationMemory.vi"("error in (no error)"=w506, "Action"=enum16{"Read", "Load", "Save"}."Read") -> ("OptionsOut"=w508:T11, "error out"=w509:errorcluster)  [unwired: 16 in]
            n197 = Unbundle By Name(w508) -> ("FlatFolderStructure"=w503:bool)
            n198 = Match Pattern(string=w515, regular expression="Interface") -> (offset past match=w513:i32)  [unwired: 1 in, 3 out]
            n199 = Greater Or Equal To 0?(x=w513) -> (x >= 0?=w512:bool)
            n200 = case shown="False" w512 {
              tunnel: [w525 w535] -> w519
              tunnel: w509 -> [w523 w535]
              tunnel: w517 -> [w522 _]
              tunnel: w503 -> [w521 _]
              frame False {
                (unwired) TRUE ("CreateThePfysicalFolderIfPossible(False)")
                n201 = Not(x=w521) -> (.not. x?=w520:bool)
                n202 = call "GDSProject_CreateFolder.vi"("Project Item To Create Folder Below(Use MyComputer if not wired)"=w522, "FolderName"="private", "error in (no error)"=w523, "CreateThePhysicalFolderIfPossible(False)"=w520) -> ("ItemOut"=w528:refnum<vi>, "FolderCreated"=w524:bool, "error out"=w526:errorcluster)  [unwired: 12 in, 1 out]
                n203 = case shown="True" w524 {
                  tunnel: w528 -> [_ w530]
                  tunnel: w526 -> [w529 w533]
                  tunnel: [w529 w531] -> w525
                  tunnel: w522 -> [_ w532]
                  frame False {
                  }
                  frame True {
                    n204 = invoke class="LVClassLibrary" method="Set Source Scope"(reference=w532, error in=w533, "SourceRef"=w530, "Scope"=T7."private" ("scope")) -> (error out=w531:errorcluster)  [unwired: 1 in, 4 out]
                    n205 = Close Reference(reference=w530, error in (no error)=w531) -> ()  [unwired: 1 out]
                  }
                }
              }
              frame True {
              }
            }
          }
          frame "CloseRefs", "Error", Default {
            n206 = case shown="\"CloseRefs\"" w558 {
              tunnel: w542 -> [w585 w592]
              tunnel: w547 -> [w584 w589]
              tunnel: [w585 w591] -> w548
              frame "False", Default {
                n207 = Unbundle By Name(w584) -> ("VIs"=w583:refnum<vi>[])
                n208 = Close Reference(reference=w583) -> ()  [unwired: 1 in, 1 out]
              }
              frame "CloseRefs" {
                n209 = Unbundle By Name(w589) -> ("ViLocked"=w590:bool[], "VIs"=w593:refnum<vi>[])
                n210 = Unbundle By Name(w589) -> ("ClassRefnum"=w588:refnum<vi>, "ClassSettings"=w587:T2)
                n211 = call "GDSLvClass_StoreClassType.vi"("Class Refnum In"=w588, "ClassSettings"=w587) -> ("error out"=w586:errorcluster)  [unwired: 16 in, 1 out]
                n212 = for {
                  tunnel: w593 -> [w598] mode=indexing
                  shift-right: [w594] -> w591
                  shift-left: w592 -> [w599]
                  tunnel: w590 -> [w595] mode=indexing
                  tunnel: w586 -> [_]
                  n213 = case shown="True" w595 {
                    tunnel: w599 -> [w603 w609]
                    tunnel: w598 -> [w604 w608]
                    tunnel: [w603 w607] -> w597
                    tunnel: [w604 w606] -> w596
                    frame False {
                    }
                    frame True {
                      n214 = invoke class="VI" method="Lock State.Set"(reference=w608, error in=w609, "lockState"=T8."Locked (No Password)" ("Lock State")) -> (reference out=w606:refnum<vi>, error out=w607:errorcluster)  [unwired: 4 in, 5 out]
                    }
                  }
                  n215 = call "Scripting_SaveVi.vi"("ForceResaving(False)"=TRUE, "error in (no error)"=w597, "VIRefToSaveIn"=w596) -> ("error out"=w602:errorcluster, "VIRefToSaveOut"=w601:refnum<vi>)  [unwired: 7 in]
                  n216 = Close Reference(reference=w601, error in (no error)=w602) -> (error out=w594:errorcluster)
                }
              }
            }
            n217 = Unbundle By Name(w547) -> ("TempClass"=w546:refnum<vi>)
            n218 = call "GOOP400_ConfigurationMemory.vi"("error in (no error)"=w542, "Action"=enum16{"Read", "Load", "Save"}."Read") -> ("OptionsOut"=w544:T11)  [unwired: 16 in, 1 out]
            n219 = Unbundle By Name(w544) -> ("FlatFolderStructure"=w540:bool)
            n220 = stacked-sequence {
              tunnel: w548 -> [w565]
              tunnel: [w565] -> w545
              tunnel: w546 -> [w566]
              frame #0 {
                n221 = Close Reference(reference=w566) -> ()  [unwired: 1 in, 1 out]
              }
            }
            n222 = Unbundle By Name(w547) -> ("DeleteFiles"=w554:path[], "App"=w550:refnum<vi>, "ProjectRefnum"=w557:refnum<vi>, "ClassRefnum"=w536:refnum<vi>)
            n223 = call "GDSLvClass_SaveEverythingInClass.vi"("ClassRefIn"=w536, "error in"=w545) -> ("error out"=w539:errorcluster)  [unwired: 16 in, 1 out]
            n224 = Close Reference(reference=w557, error in (no error)=w539) -> (error out=w551:errorcluster)
            n225 = Close Reference(reference=w550, error in (no error)=w551) -> (error out=w549:errorcluster)
            n226 = for {
              shift-right: [w581] -> w541
              shift-left: w549 -> [w582]
              tunnel: w554 -> [w580] mode=indexing
              tunnel: [w579] -> w553 mode=indexing
              n227 = Delete(path (use dialog)=w580, error in=w582) -> (error out=w581:errorcluster)  [unwired: 3 in, 2 out]
              n228 = Strip Path(path=w580) -> (stripped path=w579:path)  [unwired: 1 out]
            }
            n229 = case shown="True" w540 {
              tunnel: w541 -> [w560 w563]
              tunnel: [w560 w562] -> w538
              tunnel: w536 -> [_ w561]
              frame False {
              }
              frame True {
                n230 = call "GDSLvClass_FlattenClass.vi"("Class Refnum In"=w561, "FlattenClass(T=>Flat,F=>Not Flat)"=TRUE, "error in (no error)"=w563) -> ("error out"=w562:errorcluster)  [unwired: 15 in, 1 out]
              }
            }
            n231 = case shown="False" w552 {
              tunnel: [w569 w570] -> w537
              tunnel: w538 -> [w568 w570]
              tunnel: w536 -> [w567 _]
              frame False {
                n232 = Close Reference(reference=w567, error in (no error)=w568) -> (error out=w569:errorcluster)
              }
              frame True {
              }
            }
            n233 = for {
              tunnel: w553 -> [w575] mode=indexing
              tunnel: w537 -> [_]
              n234 = List Folder(path=w575) -> (path out=w571:path, filenames=w574:string[], error out=w572:errorcluster)  [unwired: 3 in, 1 out]
              n235 = Empty Array?(array=w574) -> (empty?=w573:bool)
              n236 = case shown="True" w573 {
                tunnel: w572 -> [_ w578]
                tunnel: w571 -> [_ w577]
                tunnel: [_ w576] -> _
                frame False {
                }
                frame True {
                  n237 = Delete(path (use dialog)=w577, error in=w578) -> (error out=w576:errorcluster)  [unwired: 3 in, 2 out]
                }
              }
            }
            n238 = call "GDSError_LogErrorInformation.vi"("State"=w555, "LocalVariableData"=w547, "error in (no error)"=w537) -> ("error out"=w556:errorcluster)  [unwired: 16 in]
          }
        }
        n239 = Equal?(x=w34, y="Exit") -> (x = y?=w38:bool)
        n240 = Select(t="Error", s=w33, f=w34) -> (s? t:f=w37:string)
      }
      n241 = Unbundle By Name(w14) -> ("ClassRefnum"=w17:refnum<vi>, "TemplateVersion"=w16:string)
    }
    frame Error {
    }
  }
  "error out" <- w11
  "LVClassLibraryRefnum" <- w4
  "TemplateVersionUsed" <- w3
  "ClassWriterGOOP400.lvclass" <- "ClassWriterGOOP400.lvclass"
